vi "Prepare Report Path.vi"(8 "error in":errorcluster, 11 "Report File Name":string="caraya-report.xml") -> (0 "error out":errorcluster, 3 "Report Path":path)   [LabVIEW 2026]
doc: "Test support for the ATM Caraya runner. Returns the absolute path of Tests\\results\\<Report File Name>, located relative to this VI (one folder up from Support), creates the results folder when it is missing and deletes a report left by an earlier run, so a report found after the run was written BY that run. A missing folder or a missing old report is not an error."
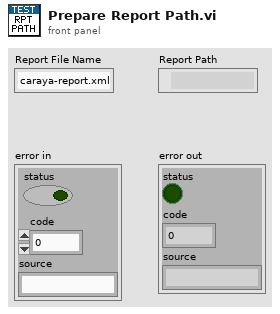
[diagram p1: front panel]
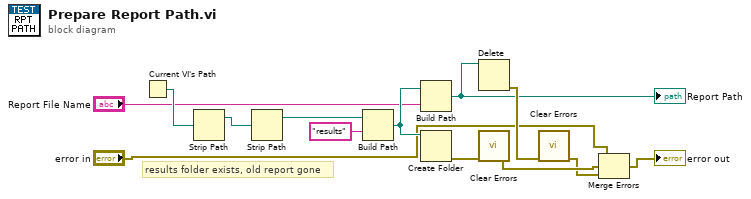
[diagram p0: block diagram]
diagram:
  # "results folder exists, old report gone"
  n1 = Current VI's Path() -> (path=w6:path)
  n2 = Strip Path(path=w6) -> (stripped path=w7:path)  [unwired: 1 out]
  n3 = Strip Path(path=w7) -> (stripped path=w8:path)  [unwired: 1 out]
  n4 = Build Path(base path=w8, name or relative path="results" ("Results Folder Name")) -> (appended path=w9:path)
  n5 = Build Path(base path=w9, name or relative path="Report File Name") -> (appended path=w4:path)
  "Report Path" <- w4
  n6 = Create Folder(path (use dialog)=w9) -> (error out=w10:errorcluster)  [unwired: 2 in, 2 out]
  n7 = Delete(path (use dialog)=w4) -> (error out=w11:errorcluster)  [unwired: 4 in, 2 out]
  n8 = call <vilib>:"Clear Errors.vi"("error in (no error)"=w10) -> ("error out"=w13:errorcluster)  [unwired: 5 in, 1 out]
  n9 = call <vilib>:"Clear Errors.vi"("error in (no error)"=w11) -> ("error out"=w12:errorcluster)  [unwired: 5 in, 1 out]
  n10 = Merge Errors("error in", w13, w12) -> (→"error out":errorcluster)
